vi "angle conversion.vi"(1 "Numeric Control":dbl format="%#_13g") -> (0 "x+y":dbl)   [LabVIEW 2019]
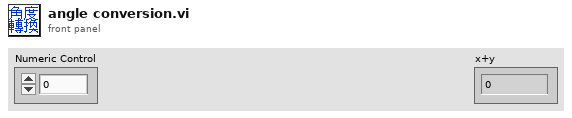
[diagram p1: front panel]
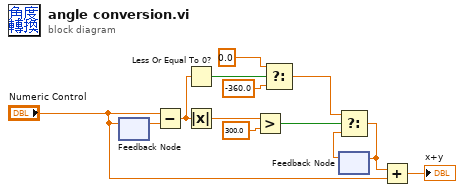
[diagram p0: block diagram]
diagram:
  n1 = feedback-in #1("Numeric Control") -> ()
  n2 = feedback #1() -> (w13:dbl)  [unwired: 1 in]
  n3 = Subtract(x="Numeric Control", y=w13) -> (x-y=w9:dbl)
  n4 = Less Or Equal To 0?(x=w9) -> (x <= 0?=w8:bool)
  n5 = Absolute Value(x=w9) -> (abs(x)=w10:dbl)
  n6 = Greater?(x=w10, y=300.0) -> (0:w11:bool)
  n7 = Select(t=0.0, s=w8, f=-360.0) -> (s? t:f=w3:dbl)
  n8 = feedback #2() -> (w1:dbl)  [unwired: 1 in]
  n9 = Select(t=w3, s=w11, f=w1) -> (s? t:f=w2:dbl)
  n10 = feedback-in #2(w2) -> ()
  n11 = Add(x=w2, y="Numeric Control") -> (x+y=→"x+y":dbl)
